vi "Get Buttons Reference.vi"(8 "error in (no error)":errorcluster, 10 "VI reference (calling)":refnum<vi>, 11 "Dialog in":refnum<class "Dialog.lvclass">) -> (0 "error out":errorcluster, 2 "VI reference (dup)":refnum<vi>, 3 "Dialog out":refnum<class "Dialog.lvclass">)   [LabVIEW 2012, in "Dialog.lvlib" / "Dialog.lvclass"]
uses:
  Dialog.lvclass
  Dialog.lvclass/Dialog.ctl
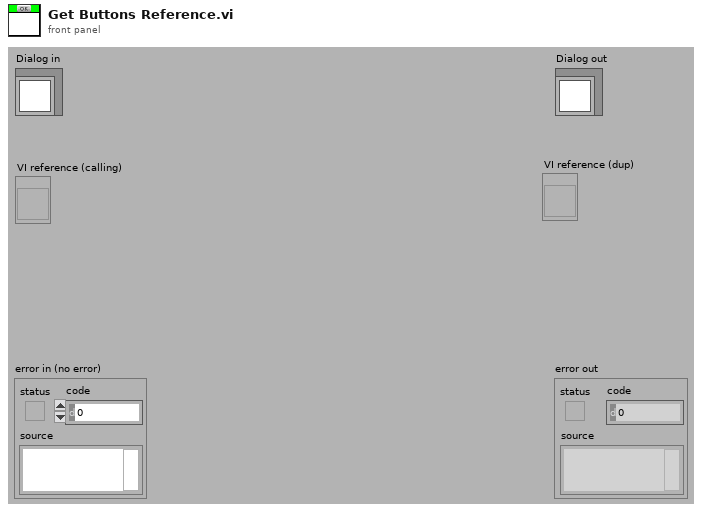
[diagram p1: front panel]
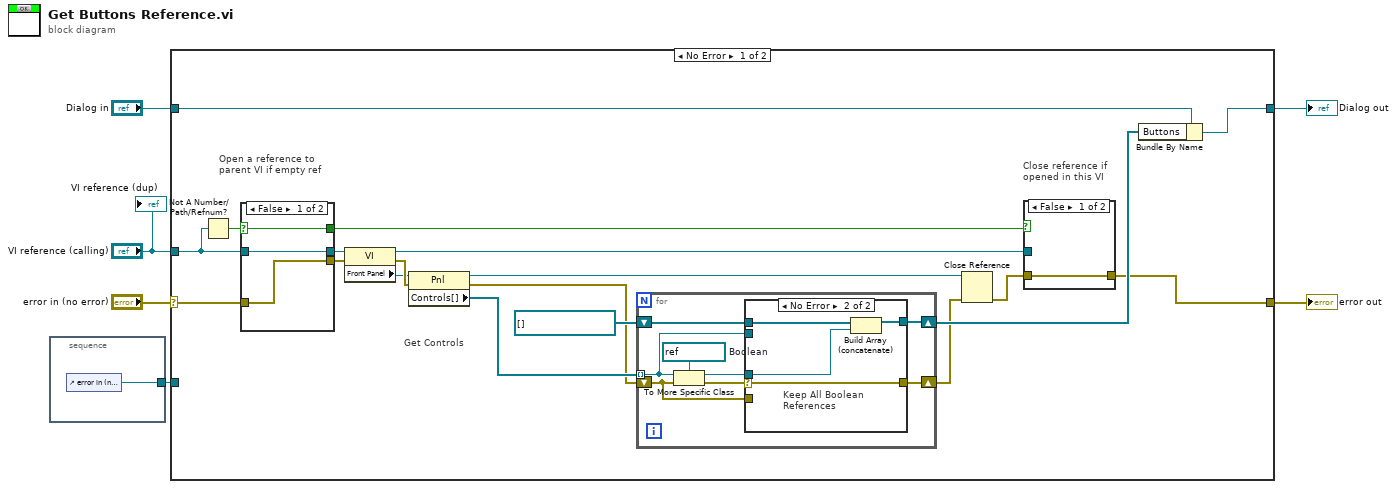
[diagram p0: block diagram]
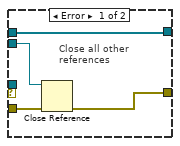
[diagram p2: hidden frame]
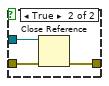
[diagram p3: hidden frame]
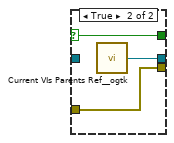
[diagram p4: hidden frame]
diagram:
  n1 = stacked-sequence {
    tunnel: [w7] -> w1
    frame #0 {
      n2 = control-ref of="error in (no error)"() -> (w7:refnum<vi>)
    }
  }
  n3 = case shown="No Error" "error in (no error)" {
    selector: "error in (no error)" -> [w19 w54]
    tunnel: [w9 w54] -> w5
    tunnel: [w23 w53] -> w3
    tunnel: "Dialog in" -> [w24 w53]
    tunnel: "VI reference (calling)" -> [w20 _]
    tunnel: w1 -> [_ _]
    frame No Error {
      # "Get Controls"
      # "Close reference if\nopened in this VI"
      # "Open a reference to\nparent VI if empty ref"
      n4 = Not A Number/Path/Refnum?(number/path/refnum=w20) -> (NaN/Path/Refnum?=w22:bool)
      n5 = case shown="False" w22 {
        selector: w22 -> [w48 w52]
        tunnel: [w48 w52] -> w17
        tunnel: [w49 w51] -> w21
        tunnel: w20 -> [w49 _]
        tunnel: w19 -> [w47 w50]
        tunnel: [w47 w50] -> w18
        frame False {
        }
        frame True {
          n6 = call <userlib>:"Current VIs Parents Ref__ogtk.vi"() -> ("Calling VI's Reference"=w51:refnum<vi>)  [unwired: 2 out]
        }
      }
      n7 = property on="Property Node" class="VI"(reference=w21, error in=w18) -> (reference out=w16:refnum<vi>, error out=w26:errorcluster, "Front Panel"=w25:refnum<vi>)
      n8 = property on="Property Node" class="Pnl"(reference=w25, error in=w26) -> (reference out=w15:refnum<vi>, error out=w8:errorcluster, "Controls[]"=w13:refnum<vi>[])
      n9 = for {
        tunnel: w13 -> [w27] mode=indexing
        shift-right: [w34] -> w12
        shift-left: refnum<vi>[] [] -> [w33]
        shift-right: [w32] -> w10
        shift-left: w8 -> [w28]
        w31 = refnum<vi> refnum  # Boolean
        n10 = To More Specific Class(target class=w31, reference=w27, error in=w28) -> (specific class reference=w29:refnum<vi>, error out=w30:errorcluster)
        n11 = case shown="No Error" w30 {
          selector: w30 -> [_ w39]
          tunnel: w29 -> [_ w40]
          tunnel: [w38 w41] -> w34
          tunnel: w33 -> [w38 w42]
          tunnel: [w36 w39] -> w32
          tunnel: w28 -> [w37 _]
          tunnel: w27 -> [w35 _]
          frame Error {
            # "Close all other\nreferences"
            n12 = Close Reference(reference=w35, error in (no error)=w37) -> (error out=w36:errorcluster)
          }
          frame No Error {
            # "Keep All Boolean\nReferences"
            n13 = Build Array (concatenate)(w42, w40) -> (w41:refnum<vi>[])
          }
        }
      }
      n14 = Close Reference(reference=w15, error in (no error)=w10) -> (error out=w14:errorcluster)
      n15 = case shown="False" w17 {
        tunnel: w16 -> [_ w46]
        tunnel: [w43 w45] -> w9
        tunnel: w14 -> [w43 w44]
        frame False {
        }
        frame True {
          n16 = Close Reference(reference=w46, error in (no error)=w44) -> (error out=w45:errorcluster)
        }
      }
      n17 = Bundle By Name(cluster=w24, "Buttons"=w12) -> (w23:refnum<class "Dialog.lvclass">)
    }
    frame Error {
    }
  }
  "error out" <- w5
  "Dialog out" <- w3
  "VI reference (dup)" <- "VI reference (calling)"
